vi "Main.vi"(10 "IP":string, 11 "Module Admin":refnum<class "Delacor_lib_QMH_Cloneable Module Admin.lvclass">) -> ()   [LabVIEW 2026, in "My Cloneable Module.lvlib"]
doc: "This template is based off of the Queued Message Handler design pattern and the Queued Message Handler project template that ships with LabVIEW.\n\nThe main difference is that the queue is private to this module and communication between modules is performed via Broadcast and Request events.\n\nRequest events are wrapped in public API methods and are handled in the Event Handling Loop (EHL) of this VI. Any module can register for Broadcast events sent by this module. The EHL generates messages based on user interface actions.\n\nThe Message Handling Loop (MHL) processes messages generated by the EHL, or by other messages. The messages are string values, so new messages can be added easily to the Message Cases case structure in the MHL. Each message cluster can also provide an optional value for Message Data, which is a variant that can be converted to whatever message-specific data is required.\n_____\nBased on DQMH Dev Tools: Project Template 7.1.2.1547."
uses:
  My Cloneable Module.lvlib
  <vilib>/Delacor/Delacor QMH/Libraries/Cloneable Module Admin_class/Delacor_lib_QMH_Cloneable Module Admin.lvclass
  C:/Program Files/National Instruments/LabVIEW 2026/vi.lib/Delacor/Delacor QMH/Libraries/Module Admin_class/Delacor_lib_QMH_Module Admin.lvclass
  Module Data--cluster.ctl
  Do Something Argument--cluster.ctl
  <vilib>/Delacor/Delacor QMH/Libraries/Cloneable Module Admin_class/Delacor_lib_QMH_Cloneable Module Admin.lvclass/Delacor_lib_QMH_Cloneable Module Admin.ctl
  <vilib>/Delacor/Delacor QMH/Libraries/Message Queue_class/Delacor_lib_QMH_Message Queue.lvclass/Delacor_lib_QMH_Message Queue.ctl
  Do Something Else Argument--cluster.ctl
  Do Something Else and Wait for Reply Argument--cluster.ctl
  Do Something Else and Wait (Reply Payload)--cluster.ctl
  Stop Argument--cluster.ctl
  <vilib>/Delacor/Delacor QMH/Libraries/Module Admin_class/Delacor_lib_QMH_Module Admin.lvclass/Delacor_lib_QMH_Module Admin.ctl
  <vilib>/Utility/miscctls.llb/LVPointTypeDef.ctl
  <vilib>/Delacor/Delacor QMH/Libraries/Message Queue_class/Delacor_lib_QMH_Enqueue Message (Single).vi
  <vilib>/Delacor/Delacor QMH/Libraries/Cloneable Module Admin_class/Delacor_lib_QMH_Get Module ID.vi
  <vilib>/Delacor/Delacor QMH/Libraries/Module Admin_class/Delacor_lib_QMH_Get External Launch.vi
  <vilib>/Delacor/Delacor QMH/Libraries/Message Queue_class/Delacor_lib_QMH_Message Queue.lvclass
panel:
  out "error out":errorcluster
  out "X":dbl
  out "Status":string
  in  "Simulate EHL Error":bool
  in  "Simulate MHL Error":bool
  in  "Do Something Else <Replace Me>":bool
  in  "Do Something <Replace Me>":bool
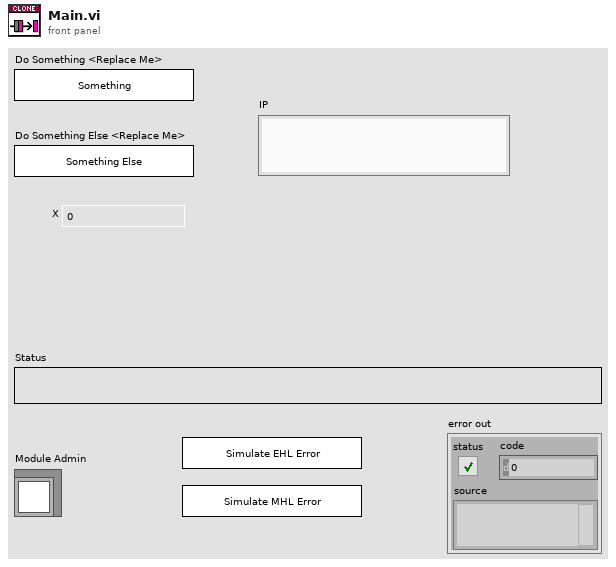
[diagram p1: front panel]
types:
  T1 = typedef "My Cloneable Module.lvlib/Request Events--cluster.ctl" = cluster{"Stop Module":refnum<user-event>, "Do Something":refnum<user-event>, "Do Something Else":refnum<user-event>, "Do Something Else and Wait for Reply":refnum<user-event>, "Show Panel":refnum<user-event>, "Hide Panel":refnum<user-event>, "Show Diagram":refnum<user-event>, "Get Module Execution Status":refnum<user-event>, "Request a HL":refnum<user-event>}
  T2 = typedef "My Cloneable Module.lvlib/Module Data--cluster.ctl" = cluster{"Status":string}
  T3 = typedef "My Cloneable Module.lvlib/Do Something Argument--cluster.ctl" = cluster{"Module ID":i32, "Do Something Msg":string}
  T4 = typedef "My Cloneable Module.lvlib/Do Something Else Argument--cluster.ctl" = cluster{"Module ID":i32, "Do Something Else Msg":string, "X":dbl}
  T5 = typedef "My Cloneable Module.lvlib/Do Something Else and Wait for Reply Argument--cluster.ctl" = cluster{"Module ID":i32, "Do Something Else Msg":string, "X":dbl, "Wait Notifier":refnum<notifier>, "wait for reply":bool}
  T6 = enum32{"invalid lock state", "Not Locked", "Locked (No Password)", "Password-protected"}
  T7 = typedef "My Cloneable Module.lvlib/Stop Argument--cluster.ctl" = cluster{"Module ID":i32, "Origin":string, "Exit via Stop Module Req?":bool, "Wait for Module to stop?":bool}
  T8 = typedef "LVPointTypeDef.ctl" = cluster{"Horizontal":i16, "Vertical":i16}
  T9 = enum32{"Invalid", "Standard", "Closed", "Hidden", "Minimized", "Maximized"}
  T10 = typedef "My Cloneable Module.lvlib/Do Something Else and Wait (Reply Payload)--cluster.ctl" = cluster{"Value":dbl, "error":errorcluster, "Module ID":i32}
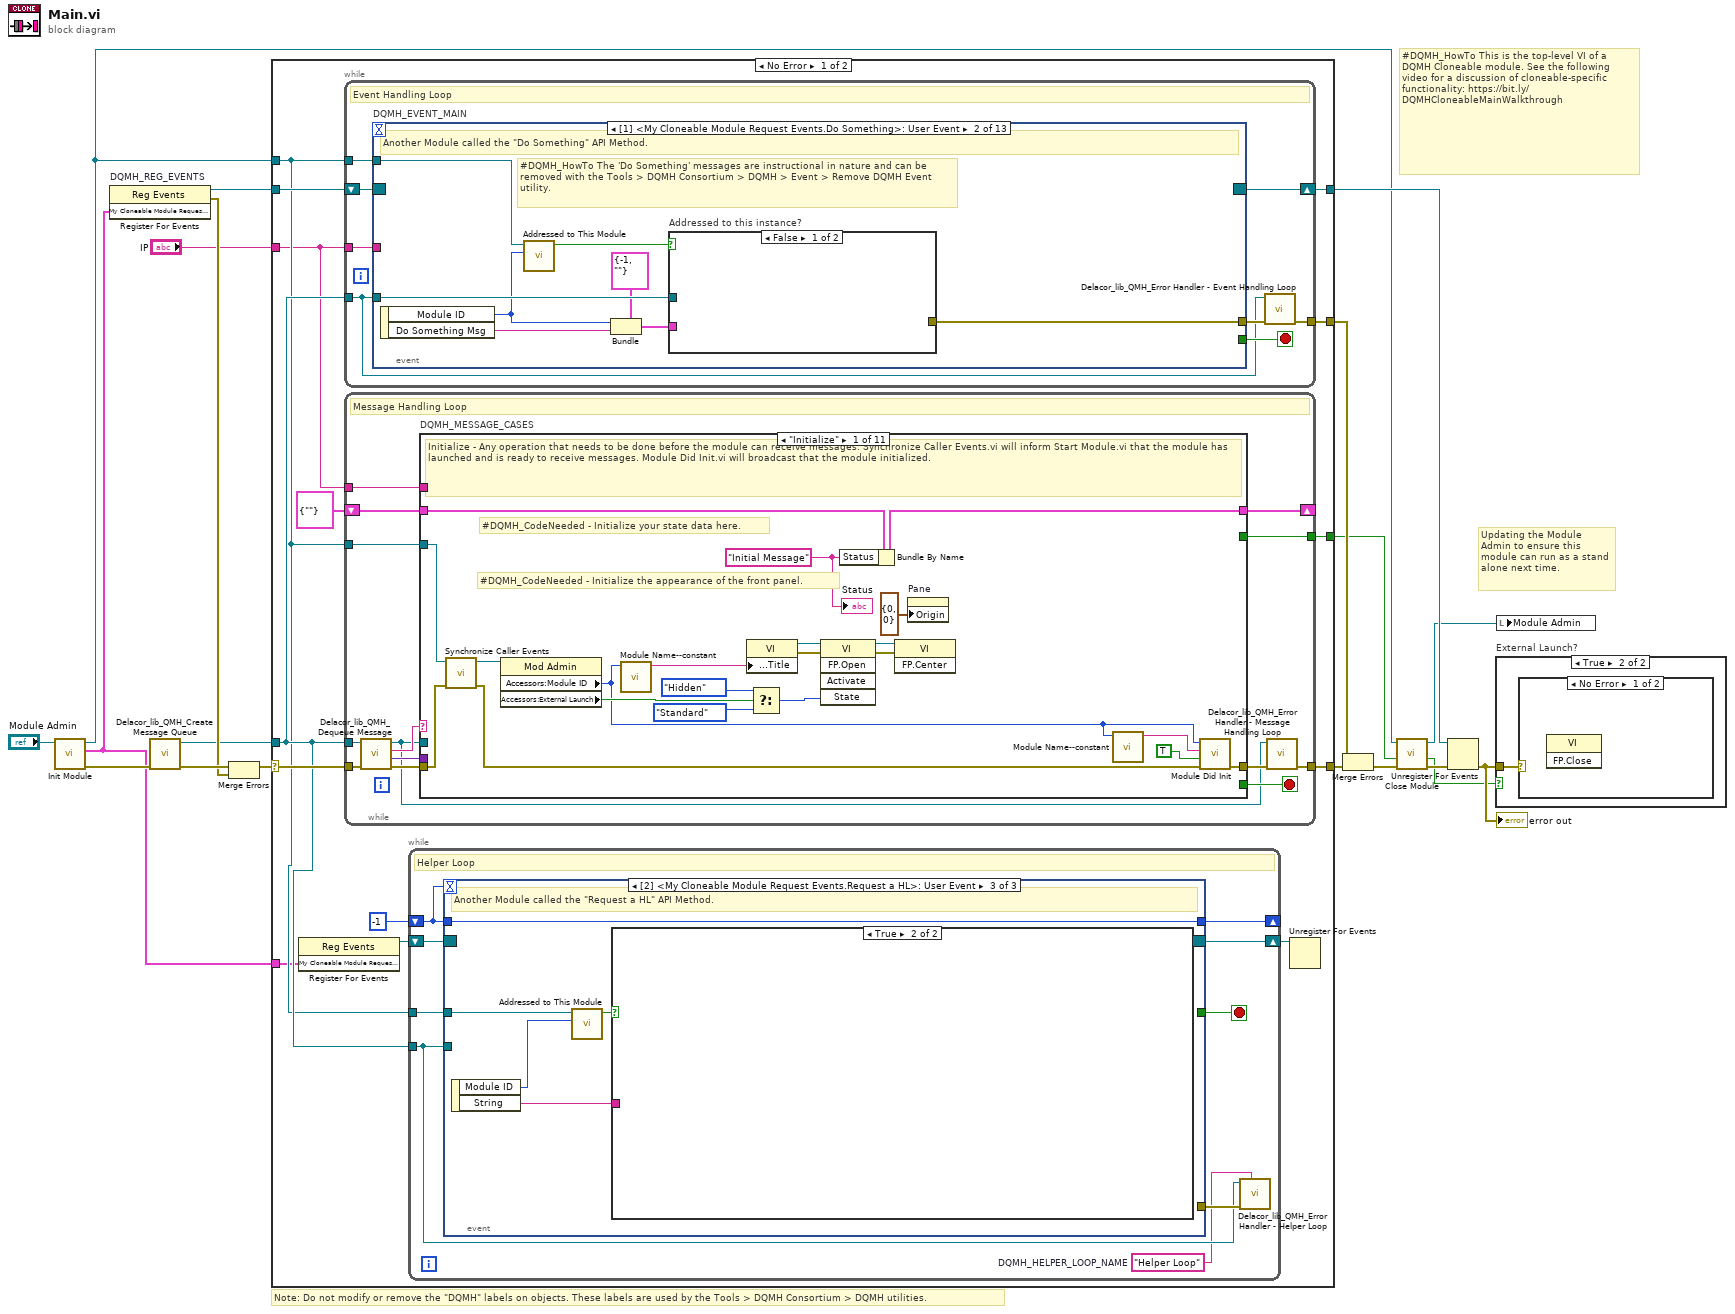
[diagram p0: block diagram]
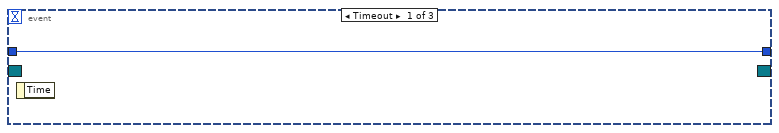
[diagram p2: hidden frame]
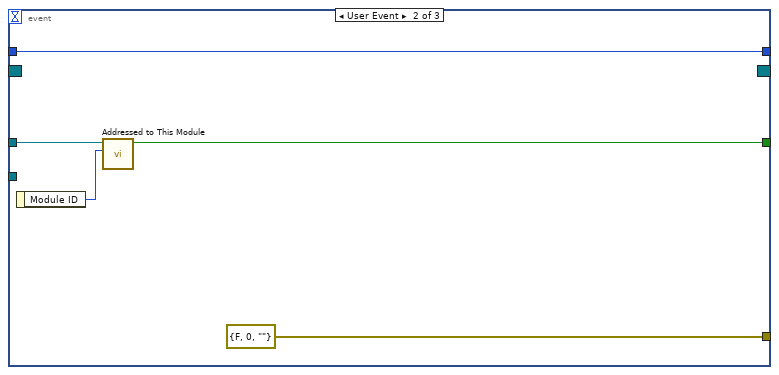
[diagram p3: hidden frame]
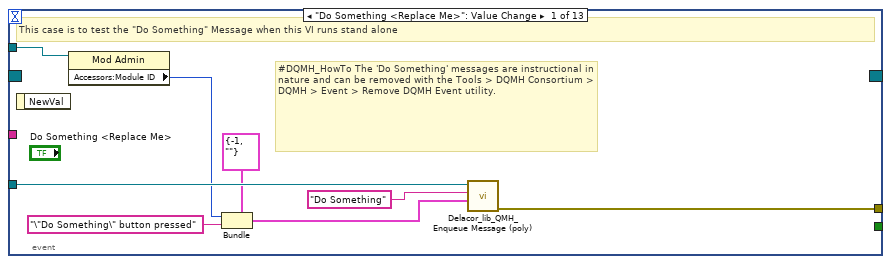
[diagram p5: hidden frame]
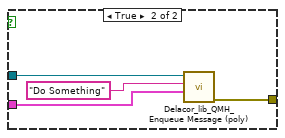
[diagram p6: hidden frame]
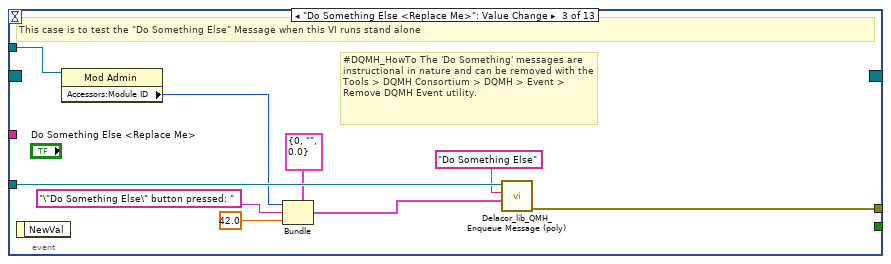
[diagram p7: hidden frame]
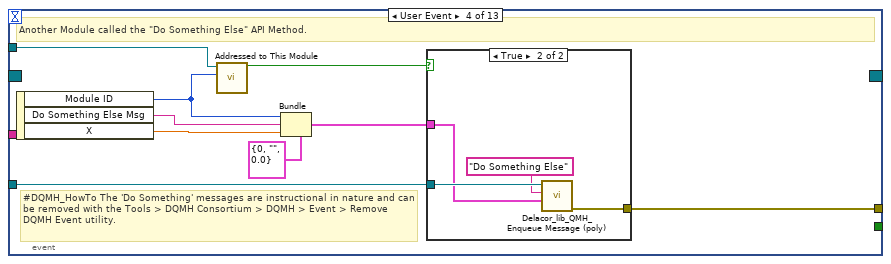
[diagram p8: hidden frame]
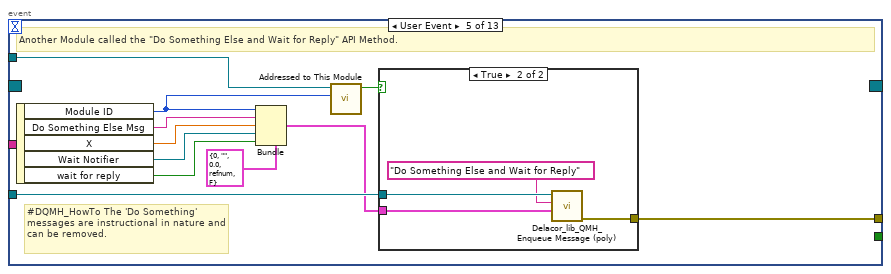
[diagram p10: hidden frame]
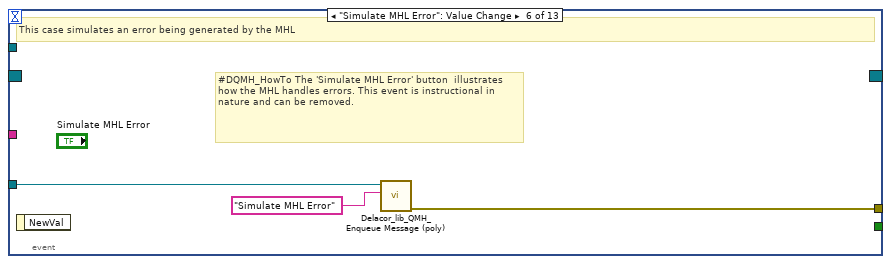
[diagram p12: hidden frame]
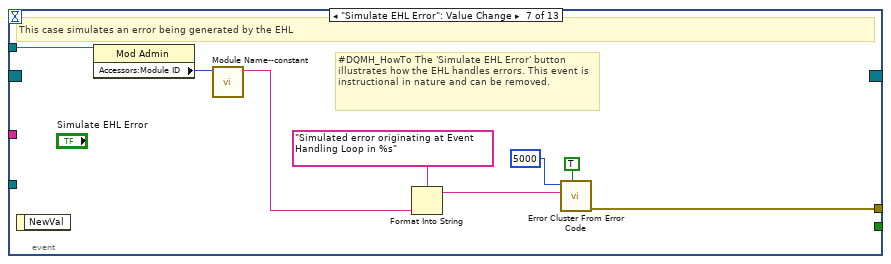
[diagram p13: hidden frame]
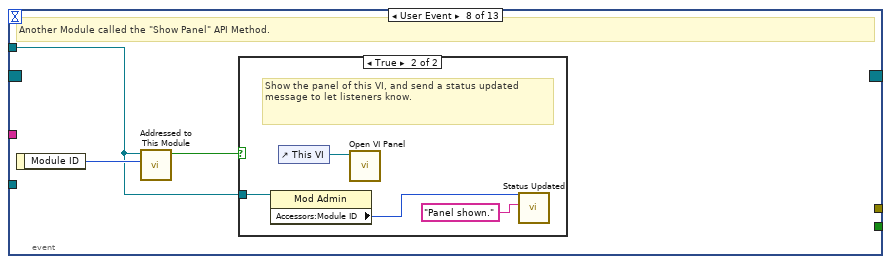
[diagram p14: hidden frame]
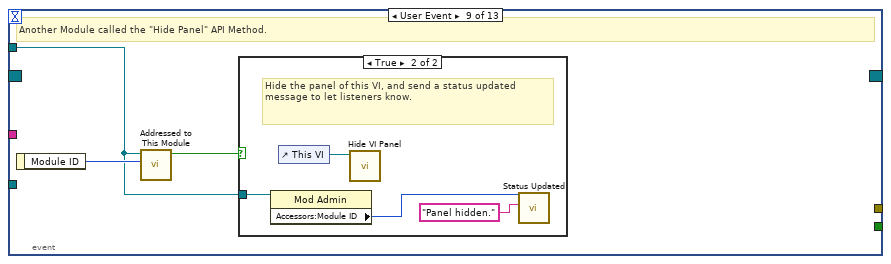
[diagram p16: hidden frame]
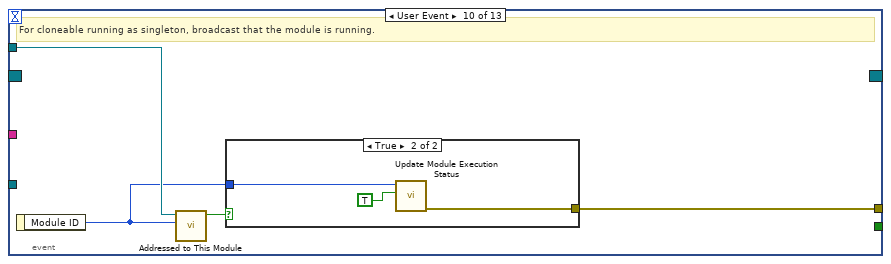
[diagram p18: hidden frame]
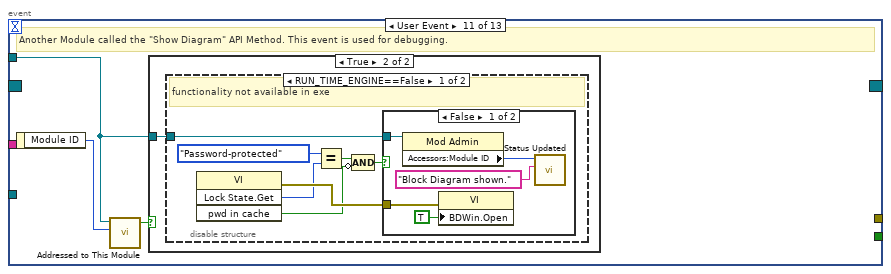
[diagram p20: hidden frame]
diagram:
  # "#DQMH_HowTo This is the top-level VI of a DQMH Cloneable module. See the following video for a discussion of cloneable-specific functionality: https://bit.ly/DQMHCloneableMainWalkthrough"
  # "Note: Do not modify or remove the \"DQMH\" labels on objects. These labels are used by the Tools > DQMH Consortium > DQMH utilities."
  # "Updating the Module Admin to ensure this module can run as a stand alone next time."
  n1 = call "Init Module.vi"("Cloneable Module Admin in"="Module Admin") -> ("error out"=w16:errorcluster, "My Cloneable Module Request Events"=w1:T1, "Cloneable Module Admin out"=w6:refnum<class "Delacor_lib_QMH_Cloneable Module Admin.lvclass">)  [unwired: 8 in]
  n2 = register-events "DQMH_REG_EVENTS"(w1) -> (reference out=w9:refnum<event-registration>, error out=w11:errorcluster)  [unwired: 2 in]
  n3 = call <vilib>:"Delacor_lib_QMH_Create Message Queue.vi"("error in"=w16) -> ("error out"=w13:errorcluster, "Message Queue"=w8:refnum<class "Delacor_lib_QMH_Message Queue.lvclass">)  [unwired: 9 in]
  n4 = Merge Errors(w13, w11) -> (w12:errorcluster)
  n5 = case shown="No Error" w12 {
    selector: w12 -> [w31 w364]
    tunnel: [w33 w363] -> w17
    tunnel: [w30 w362] -> w10
    tunnel: w9 -> [w28 w362]
    tunnel: w8 -> [w27 w355]
    tunnel: [w32 _] -> w18
    tunnel: w6 -> [w26 w358]
    tunnel: [w25 _] -> w4
    tunnel: "IP" -> [w24 _]
    tunnel: w1 -> [w23 _]
    frame No Error {
      n6 = register-events ("DQMH_HELPER_REGFOREVENTS")(w23) -> (reference out=w21:refnum<event-registration>)  [unwired: 2 in, 1 out]
      n7 = while {
        tunnel: w27 -> [w55]
        shift-right: [w58] -> w30
        shift-left: w28 -> [w59]
        tunnel: [w60] -> w32
        tunnel: w26 -> [w56]
        tunnel: w24 -> [w54]
        stop <- w57 stop-if-true
        # "Event Handling Loop"
        n8 = event "DQMH_EVENT_MAIN" shown="[1] <My Cloneable Module Request Events.Do Something>: User Event" {
          selector: w59 -> [_ _ _ _ _ _ _ _ _ _ _ _ _]
          dyn-events: [_ _ _ _ _ _ _ _ _ _ _ _ _] -> w58
          timeout: _ -> [_ _ _ _ _ _ _ _ _ _ _ _ _]
          tunnel: [_ _ _ _ _ _ _ _ _ _ _ w170 _] -> w57
          tunnel: w55 -> [w68 w76 w89 w98 w113 w120 _ _ _ _ _ w173 w190]
          tunnel: [w69 w77 w90 w99 w114 w121 w129 _ _ w147 _ w174 w193] -> w61
          tunnel: w56 -> [w64 w74 w83 w96 w111 _ w128 w130 w137 w145 w151 w172 w191]
          tunnel: w54 -> [_ _ _ _ _ _ _ _ _ _ _ _ _]
          event "Do Something <Replace Me>": Value Change {
            # "#DQMH_HowTo The 'Do Something' messages are instructional in nature and can be removed with the Tools > DQMH Consortium > DQMH > Event > Remove DQMH Event utility."
            # "This case is to test the \"Do Something\" Message when this VI runs stand alone"
            n9 = event-data() -> ()  [unwired: 1 in, 1 out]
            n10 = property on="Property Node" class="Mod Admin"(reference=w64) -> ("Accessors:Module ID"=w63:i32)  [unwired: 1 in, 2 out]
            n11 = Bundle(cluster=T3 {"Module ID"=-1, "Do Something Msg"=""} ("Do Something Argument"), "Module ID"=w63, "Do Something Msg"="\"Do Something\" button pressed" ("\"Do Something\" button pressed")) -> (w66:T3)
            n12 = call-poly <vilib>:"Delacor_lib_QMH_Enqueue Message (poly).vi"("Message Data"=w66, "Message"="Do Something", "Message Queue in"=w68) -> ("error out"=w69:errorcluster)  [unwired: 7 in, 1 out]
          }
          event User Event {
            # "#DQMH_HowTo The 'Do Something' messages are instructional in nature and can be removed with the Tools > DQMH Consortium > DQMH > Event > Remove DQMH Event utility."
            # "Another Module called the \"Do Something\" API Method."
            n13 = event-data() -> ("Module ID"=w71:i32, "Do Something Msg"=w70:string)  [unwired: 1 in]
            n14 = call "Addressed to This Module.vi"("Module ID from Argument"=w71, "Module Admin"=w74) -> ("Addressed to this instance?"=w75:bool)  [unwired: 8 in, 1 out]
            n15 = Bundle(cluster=T3 {"Module ID"=-1, "Do Something Msg"=""} ("Do Something Argument"), "Module ID"=w71, "Do Something Msg"=w70) -> (w73:T3)
            n16 = case "Addressed to this instance?" shown="False" w75 {
              tunnel: w76 -> [_ w80]
              tunnel: [_ w81] -> w77
              tunnel: w73 -> [_ w78]
              frame False {
                # "Do nothing"
              }
              frame True {
                n17 = call-poly <vilib>:"Delacor_lib_QMH_Enqueue Message (poly).vi"("Message Data"=w78, "Message"="Do Something", "Message Queue in"=w80) -> ("error out"=w81:errorcluster)  [unwired: 7 in, 1 out]
              }
            }
          }
          event "Do Something Else <Replace Me>": Value Change {
            # "#DQMH_HowTo The 'Do Something' messages are instructional in nature and can be removed with the Tools > DQMH Consortium > DQMH > Event > Remove DQMH Event utility."
            # "This case is to test the \"Do Something Else\" Message when this VI runs stand alone"
            n18 = event-data() -> ()  [unwired: 1 in, 1 out]
            n19 = property on="Property Node" class="Mod Admin"(reference=w83) -> ("Accessors:Module ID"=w82:i32)  [unwired: 1 in, 2 out]
            n20 = Bundle(cluster=T4 {"Module ID"=0, "Do Something Else Msg"="", "X"=0.0} ("Do Something Else Argument"), "Module ID"=w82, "Do Something Else Msg"="\"Do Something Else\" button pressed: " ("\"Do Something Else\" button pressed"), "X"=42.0) -> (w86:T4)
            n21 = call-poly <vilib>:"Delacor_lib_QMH_Enqueue Message (poly).vi"("Message Data"=w86, "Message"="Do Something Else", "Message Queue in"=w89) -> ("error out"=w90:errorcluster)  [unwired: 7 in, 1 out]
          }
          event User Event {
            # "#DQMH_HowTo The 'Do Something' messages are instructional in nature and can be removed with the Tools > DQMH Consortium > DQMH > Event > Remove DQMH Event utility."
            # "Another Module called the \"Do Something Else\" API Method."
            n22 = event-data() -> ("Module ID"=w91:i32, "Do Something Else Msg"=w92:string, "X"=w94:dbl)  [unwired: 1 in]
            n23 = call "Addressed to This Module.vi"("Module ID from Argument"=w91, "Module Admin"=w96) -> ("Addressed to this instance?"=w97:bool)  [unwired: 8 in, 1 out]
            n24 = Bundle(cluster=T4 {"Module ID"=0, "Do Something Else Msg"="", "X"=0.0} ("Do Something Else Argument"), "Module ID"=w91, "Do Something Else Msg"=w92, "X"=w94) -> (w93:T4)
            n25 = case shown="True" w97 {
              tunnel: w98 -> [_ w102]
              tunnel: [_ w103] -> w99
              tunnel: w93 -> [_ w100]
              frame False {
              }
              frame True {
                n26 = call-poly <vilib>:"Delacor_lib_QMH_Enqueue Message (poly).vi"("Message Data"=w100, "Message"="Do Something Else", "Message Queue in"=w102) -> ("error out"=w103:errorcluster)  [unwired: 7 in, 1 out]
              }
            }
          }
          event User Event {
            # "#DQMH_HowTo The 'Do Something' messages are instructional in nature and can be removed."
            # "Another Module called the \"Do Something Else and Wait for Reply\" API Method."
            n27 = event-data() -> ("Module ID"=w109:i32, "Do Something Else Msg"=w107:string, "X"=w106:dbl, "Wait Notifier"=w105:refnum<notifier>, "wait for reply"=w104:bool)  [unwired: 1 in]
            n28 = Bundle(cluster=T5 {"Module ID"=0, "Do Something Else Msg"="", "X"=0.0, "Wait Notifier"=refnum, "wait for reply"=FALSE} ("Do Something Else and Wait for Reply Argument"), "Module ID"=w109, "Do Something Else Msg"=w107, "X"=w106, "Wait Notifier"=w105, "wait for reply"=w104) -> (w108:T5)
            n29 = call "Addressed to This Module.vi"("Module ID from Argument"=w109, "Module Admin"=w111) -> ("Addressed to this instance?"=w112:bool)  [unwired: 8 in, 1 out]
            n30 = case shown="True" w112 {
              tunnel: [_ w118] -> w114
              tunnel: w113 -> [_ w117]
              tunnel: w108 -> [_ w115]
              frame False {
              }
              frame True {
                n31 = call-poly <vilib>:"Delacor_lib_QMH_Enqueue Message (poly).vi"("Message Data"=w115, "Message"="Do Something Else and Wait for Reply", "Message Queue in"=w117) -> ("error out"=w118:errorcluster)  [unwired: 7 in, 1 out]
              }
            }
          }
          event "Simulate MHL Error": Value Change {
            # "#DQMH_HowTo The 'Simulate MHL Error' button  illustrates how the MHL handles errors. This event is instructional in nature and can be removed."
            # "This case simulates an error being generated by the MHL"
            n32 = event-data() -> ()  [unwired: 1 in, 1 out]
            n33 = call-poly <vilib>:"Delacor_lib_QMH_Enqueue Message (poly).vi"("Message"="Simulate MHL Error", "Message Queue in"=w120) -> ("error out"=w121:errorcluster)  [unwired: 8 in, 1 out]
          }
          event "Simulate EHL Error": Value Change {
            # "#DQMH_HowTo The 'Simulate EHL Error' button  illustrates how the EHL handles errors. This event is instructional in nature and can be removed."
            # "This case simulates an error being generated by the EHL"
            n34 = event-data() -> ()  [unwired: 1 in, 1 out]
            n35 = property on="Property Node" class="Mod Admin"(reference=w128) -> ("Accessors:Module ID"=w127:i32)  [unwired: 1 in, 2 out]
            n36 = call "Module Name--constant.vi"("Module ID"=w127) -> ("Module Name"=w122:string)  [unwired: 10 in]
            n37 = Format Into String(format string="Simulated error originating at Event Handling Loop in %s", w122) -> (resulting string=w125:string)  [unwired: 2 in, 1 out]
            n38 = call <vilib>:"Error Cluster From Error Code.vi"("show call chain? (False)"=TRUE, "error message (\"\")"=w125, "error code (0)"=5000) -> ("error out"=w129:errorcluster)  [unwired: 6 in]
          }
          event User Event {
            # "Another Module called the \"Show Panel\" API Method."
            n39 = event-data() -> ("Module ID"=w131:i32)  [unwired: 1 in]
            n40 = call "Addressed to This Module.vi"("Module ID from Argument"=w131, "Module Admin"=w130) -> ("Addressed to this instance?"=w132:bool)  [unwired: 8 in, 1 out]
            n41 = case shown="True" w132 {
              tunnel: w130 -> [_ w134]
              frame False {
              }
              frame True {
                # "Show the panel of this VI, and send a status updated message to let listeners know."
                n42 = property on="Property Node" class="Mod Admin"(reference=w134) -> ("Accessors:Module ID"=w133:i32)  [unwired: 1 in, 2 out]
                n43 = control-ref of="This VI"() -> (w136:refnum<vi>)
                n44 = call "Open VI Panel.vi"("VI"=w136) -> ()  [unwired: 10 in, 1 out]
                n45 = call "Status Updated.vi"("Status"="Panel shown." ("format string"), "Module ID"=w133) -> ()  [unwired: 9 in, 1 out]
              }
            }
          }
          event User Event {
            # "Another Module called the \"Hide Panel\" API Method."
            n46 = event-data() -> ("Module ID"=w138:i32)  [unwired: 1 in]
            n47 = call "Addressed to This Module.vi"("Module ID from Argument"=w138, "Module Admin"=w137) -> ("Addressed to this instance?"=w139:bool)  [unwired: 8 in, 1 out]
            n48 = case shown="True" w139 {
              tunnel: w137 -> [_ w141]
              frame False {
              }
              frame True {
                # "Hide the panel of this VI, and send a status updated message to let listeners know."
                n49 = property on="Property Node" class="Mod Admin"(reference=w141) -> ("Accessors:Module ID"=w140:i32)  [unwired: 1 in, 2 out]
                n50 = control-ref of="This VI"() -> (w143:refnum<vi>)
                n51 = call "Hide VI Panel.vi"("VI"=w143) -> ()  [unwired: 10 in, 1 out]
                n52 = call "Status Updated.vi"("Status"="Panel hidden." ("format string"), "Module ID"=w140) -> ()  [unwired: 9 in, 1 out]
              }
            }
          }
          event User Event {
            # "For cloneable running as singleton, broadcast that the module is running."
            n53 = event-data() -> ("Module ID"=w144:i32)  [unwired: 1 in]
            n54 = call "Addressed to This Module.vi"("Module ID from Argument"=w144, "Module Admin"=w145) -> ("Addressed to this instance?"=w146:bool)  [unwired: 8 in, 1 out]
            n55 = case shown="True" w146 {
              tunnel: [_ w150] -> w147
              tunnel: w144 -> [_ w149]
              frame False {
              }
              frame True {
                n56 = call "Update Module Execution Status.vi"("Running?"=TRUE, "Module ID"=w149) -> ("error out"=w150:errorcluster)  [unwired: 9 in]
              }
            }
          }
          event User Event {
            # "Another Module called the \"Show Diagram\" API Method. This event is used for debugging."
            n57 = event-data() -> ("Module ID"=w152:i32)  [unwired: 1 in]
            n58 = call "Addressed to This Module.vi"("Module ID from Argument"=w152, "Module Admin"=w151) -> ("Addressed to this instance?"=w153:bool)  [unwired: 8 in, 1 out]
            n59 = case shown="True" w153 {
              tunnel: w151 -> [_ w154]
              frame False {
              }
              frame True {
                n60 = disable-structure shown="RUN_TIME_ENGINE==False" {
                  disable-tunnel: w154 -> [w155 _]
                  frame condition #0 (active) {
                    # "functionality not available in exe"
                    n61 = invoke on="Invoke Node" class="VI" method="Lock State.Get"() -> (error out=w161:errorcluster, "Get Lock State"=w160:T6, "pwd in cache"=w157:bool)  [unwired: 4 in, 1 out]
                    n62 = Equal?(x=T6."Password-protected", y=w160) -> (x = y?=w158:bool)
                    n63 = Compound Arithmetic op=AND(w158, invert w157) -> (w156:bool)
                    n64 = case shown="False" w156 {
                      tunnel: w161 -> [w166 _]
                      tunnel: w155 -> [w163 _]
                      frame False {
                        n65 = property on="Property Node" class="Mod Admin"(reference=w163) -> ("Accessors:Module ID"=w162:i32)  [unwired: 1 in, 2 out]
                        n66 = property on="Property Node" class="VI"(error in=w166, "BDWin.Open"=TRUE ("Block Diagram Window:Open")) -> ()  [unwired: 1 in, 2 out]
                        n67 = call "Status Updated.vi"("Status"="Block Diagram shown." ("format string"), "Module ID"=w162) -> ()  [unwired: 9 in, 1 out]
                      }
                      frame True {
                        # "Password-protected VI, and the password is not in the cache. Do not show the diagram."
                      }
                    }
                  }
                  frame condition #1 {
                  }
                }
              }
            }
          }
          event User Event {
            # "Another Module called the \"Stop Module\" API Method  or the Message Handling Loop below."
            n68 = event-data() -> ("Module ID"=w168:i32, "Wait for Module to stop?"=w169:bool, "Origin"=w167:string)  [unwired: 1 in]
            n69 = call "Addressed to This Module.vi"("Module ID from Argument"=w168, "Module Admin"=w172) -> ("Addressed to this instance?"=w171:bool)  [unwired: 8 in, 1 out]
            n70 = case shown="True" w171 {
              tunnel: [_ w186] -> w174
              tunnel: w173 -> [_ w182]
              tunnel: [_ TRUE] -> w170
              tunnel: w169 -> [_ w177]
              tunnel: w168 -> [_ w179]
              tunnel: w167 -> [_ w175]
              frame False {
              }
              frame True {
                # "The event can get fired from the Exit message. The queue gets destroyed there. In this case, the Enqueue VI will return error 1. It is safe to ignore, because the module is already exiting."
                n71 = local write "Status"(w175) -> ()
                n72 = Bundle By Name(cluster=T7 {"Module ID"=-1, "Origin"="", "Exit via Stop Module Req?"=FALSE, "Wait for Module to stop?"=FALSE} ("Stop Argument"), "Module ID"=w179, "Exit via Stop Module Req?"=TRUE, "Wait for Module to stop?"=w177) -> (w176:T7)
                n73 = call-poly <vilib>:"Delacor_lib_QMH_Enqueue Message (poly).vi"("Priority Message? (F)"=TRUE, "Message Data"=w176, "Message"="Exit", "Message Queue in"=w182) -> ("error out"=w187:errorcluster)  [unwired: 6 in, 1 out]
                n74 = call <vilib>:"Clear Errors.vi"("error in (no error)"=w187, "specific error code to clear (0: all)"=1) -> ("error out"=w186:errorcluster)  [unwired: 4 in, 1 out]
              }
            }
          }
          event Panel Close? {
            w192 = TRUE  # Discard the event, the MHL is responsible for closing and stopping this VI.
            # "Hide the panel or send the 'Exit' message if the user clicks the 'X' on the module main VI panel."
            n75 = event-data() -> ()  [unwired: 1 in, 1 out]
            n76 = property on="Property Node" class="Mod Admin"(reference=w191) -> (reference out=w188:refnum<class "Delacor_lib_QMH_Cloneable Module Admin.lvclass">, "Accessors:External Launch"=w189:bool)  [unwired: 1 in, 1 out]
            n77 = case shown="True" w189 {
              tunnel: w190 -> [_ w201]
              tunnel: [_ w202] -> w193
              tunnel: w188 -> [w196 _]
              frame True {
                # "If externally launched, clicking the 'X' hides the panel, but doesn't close it."
                n78 = property on="Property Node" class="Mod Admin"(reference=w196) -> ("Accessors:Module ID"=w195:i32)  [unwired: 1 in, 2 out]
                n79 = call "Status Updated.vi"("Status"="Panel hidden." ("format string"), "Module ID"=w195) -> ("error out"=w194:errorcluster)  [unwired: 9 in]
                n80 = control-ref of="This VI"() -> (w198:refnum<vi>)
                n81 = call "Hide VI Panel.vi"("error in"=w194, "VI"=w198) -> ()  [unwired: 9 in, 1 out]
              }
              frame False {
                # "If run as a stand-alone VI, clicking the panel 'X' stops the VI."
                n82 = call-poly <vilib>:"Delacor_lib_QMH_Enqueue Message (poly).vi"("Priority Message? (F)"=TRUE, "Message"="Exit", "Message Queue in"=w201) -> ("error out"=w202:errorcluster)  [unwired: 7 in, 1 out]
              }
            }
            n83 = event-data ("Event Filter Node")("Discard?"=w192) -> ()  [unwired: 1 in, 1 out]
          }
        }
        n84 = call-dynamic "Delacor_lib_QMH_Error Handler - Event Handling Loop.vi"("error in"=w61, "Message Queue in"=w55) -> ("dup error in"=w60:errorcluster)  [unwired: 8 in, 1 out]
      }
      n85 = while {
        tunnel: w27 -> [w204]
        shift-right: [w211] -> _
        shift-left: T2 {"Status"=""} ("Data Cluster") -> [w212]
        tunnel: w31 -> [w215]
        tunnel: [w213] -> w33
        tunnel: w26 -> [w206]
        tunnel: [w205] -> w25
        tunnel: w24 -> [w203]
        stop <- w210 stop-if-true
        # "Message Handling Loop"
        n86 = call-dynamic "Delacor_lib_QMH_Dequeue Message.vi"("error in"=w215, "Message Queue in"=w204) -> ("error out"=w214:errorcluster, "Message Data"=w208:variant, "Message"=w209:string, "Message Queue out"=w207:refnum<class "Delacor_lib_QMH_Message Queue.lvclass">)  [unwired: 6 in]
        n87 = case "DQMH_MESSAGE_CASES" shown="\"Initialize\"" w209 {
          selector: w209 -> [_ _ _ _ _ _ _ _ _ _ w344]
          tunnel: w207 -> [_ _ _ _ _ _ _ w299 _ w336 _]
          tunnel: w214 -> [w235 w239 w249 w260 w281 w294 w296 w308 w325 w342 w353]
          tunnel: [w233 w239 w247 w259 w280 w293 w296 w304 w324 w337 w354] -> w216
          tunnel: w212 -> [w226 w238 w246 w258 w261 w292 w295 w303 w322 w335 w351]
          tunnel: [w225 w238 w246 w258 w261 w292 w295 w303 w322 w335 w351] -> w211
          tunnel: [_ _ _ _ _ _ _ _ _ w334 _] -> w210
          tunnel: w208 -> [_ _ w245 w255 w275 _ _ w302 _ w332 _]
          tunnel: w206 -> [w221 _ w241 w251 w266 _ _ w301 w320 w327 w350]
          tunnel: [_ _ _ _ _ _ _ _ _ w330 _] -> w205
          tunnel: w203 -> [_ _ _ _ _ _ _ _ _ _ _]
          frame "Initialize" {
            w218 = "Initial Message" ("Initial Message")
            # "#DQMH_CodeNeeded - Initialize the appearance of the front panel."
            # "#DQMH_CodeNeeded - Initialize your state data here."
            # "Initialize - Any operation that needs to be done before the module can receive messages. Synchronize Caller Events.vi will inform Start Module.vi that the module has launched and is ready to receive messages. Module Did Init.vi will broadcast that the module initialized."
            n88 = call "Synchronize Caller Events.vi"("error in"=w235, "Module Admin"=w221) -> ("error out"=w234:errorcluster, "Module Admin out"=w220:refnum<class "Delacor_lib_QMH_Cloneable Module Admin.lvclass">)  [unwired: 8 in]
            n89 = property on="Property Node" class="Mod Admin"(reference=w220) -> ("Accessors:Module ID"=w217:i32, "Accessors:External Launch"=w222:bool)  [unwired: 1 in, 2 out]
            n90 = call "Module Name--constant.vi"("Module ID"=w217) -> ("Module Name"=w230:string)  [unwired: 10 in]
            n91 = property on="Property Node" class="VI"("Front Panel.Title"=w230) -> (reference out=w232:refnum<vi>, error out=w237:errorcluster)  [unwired: 2 in]
            n92 = Select(t=T9."Hidden" ("State"), s=w222, f=T9."Standard" ("State")) -> (s? t:f=w227:T9)
            n93 = invoke on="Invoke Node" class="VI" method="FP.Open"(reference=w232, error in=w237, "State"=w227) -> (reference out=w231:refnum<vi>, error out=w236:errorcluster)  [unwired: 2 in, 3 out]
            n94 = Bundle By Name(cluster=w226, "Status"=w218) -> (w225:T2)
            n95 = invoke on="Invoke Node" class="VI" method="FP.Center"(reference=w231, error in=w236) -> ()  [unwired: 1 in, 3 out]
            n96 = property on="Pane" class="Pane"("Origin"=T8 {"Horizontal"=0, "Vertical"=0}) -> ()  [unwired: 2 in, 2 out]
            n97 = call "Module Name--constant.vi"("Module ID"=w217) -> ("Module Name"=w223:string)  [unwired: 10 in]
            n98 = call "Module Did Init.vi"("error in"=w234, "Initialized?"=TRUE, "Origin"=w223, "Module ID"=w217) -> ("error out"=w233:errorcluster)  [unwired: 7 in]
            "Status" <- w218
          }
          frame "---Module Specific---" {
            # "Separator -- The following cases handle messages specific to this Module."
          }
          frame "Do Something" {
            # "#DQMH_HowTo The 'Do Something' messages are instructional in nature and can be removed with the Tools > DQMH Consortium > DQMH > Event > Remove DQMH Event utility."
            # "Do Something - Replace this message with functionality for your own application. Note that this message also fires the \"Did Something\" broadcast event."
            n99 = Variant To Data(error in=w249, type=T3 {"Module ID"=-1, "Do Something Msg"=""} ("Do Something Argument"), Variant=w245) -> (data=w244:T3, error out=w248:errorcluster)
            n100 = property on="Property Node" class="Mod Admin"(reference=w241) -> ("Accessors:Module ID"=w240:i32)  [unwired: 1 in, 2 out]
            n101 = Unbundle By Name(w244) -> ("Do Something Msg"=w242:string)
            n102 = call "Status Updated.vi"("Status"=w242, "Module ID"=w240) -> ()  [unwired: 9 in, 1 out]
            n103 = local write "Status"(w242) -> ()
            n104 = call "Did Something.vi"("error in"=w248, "Did Something Msg"=w242, "Module ID"=w240) -> ("error out"=w247:errorcluster)  [unwired: 8 in]
          }
          frame "Do Something Else" {
            # "#DQMH_HowTo The 'Do Something' messages are instructional in nature and can be removed with the Tools > DQMH Consortium > DQMH > Event > Remove DQMH Event utility."
            # "Do Something Else - Replace this message with functionality for your own application."
            n105 = Variant To Data(error in=w260, type=T4 {"Module ID"=0, "Do Something Else Msg"="", "X"=0.0} ("Do Something Else Argument"), Variant=w255) -> (data=w256:T4, error out=w259:errorcluster)
            n106 = Unbundle By Name(w256) -> ("Do Something Else Msg"=w254:string, "X"=w253:dbl)
            "X" <- w253
            n107 = property on="Property Node" class="Mod Admin"(reference=w251) -> ("Accessors:Module ID"=w250:i32)  [unwired: 1 in, 2 out]
            n108 = Format Into String(initial string=w254, w253) -> (resulting string=w252:string)  [unwired: 2 in, 1 out]
            n109 = call "Status Updated.vi"("Status"=w252, "Module ID"=w250) -> ()  [unwired: 9 in, 1 out]
            n110 = local write "Status"(w252) -> ()
          }
          frame "Do Something Else and Wait for Reply" {
            w268 = "X(%.2f)+Offset(%.2f)=%.2f"  # status message format string
            # "#DQMH_HowTo The 'Do Something' messages are instructional in nature and can be removed."
            # "Send back X with a random offset"
            # "Do Something Else and Wait for Reply - Replace this message with functionality for your own application. Note that this message must fire a notifier to let callers know it has finished execution, and it returns an error if the 'Value' is negative."
            n111 = property on="Property Node" class="Mod Admin"(reference=w266) -> ("Accessors:Module ID"=w263:i32)  [unwired: 1 in, 2 out]
            n112 = Variant To Data(error in=w281, type=T5 {"Module ID"=0, "Do Something Else Msg"="", "X"=0.0, "Wait Notifier"=refnum, "wait for reply"=FALSE} ("Do Something Else and Wait for Reply Argument"), Variant=w275) -> (data=w276:T5, error out=w279:errorcluster)
            n113 = Unbundle By Name(w276) -> ("Wait Notifier"=w273:refnum<notifier>, "Do Something Else Msg"=w274:string, "X"=w270:dbl, "wait for reply"=w264:bool)
            n114 = Random Number (0-1)() -> (number: 0 to 1=w269:dbl)
            n115 = Add(x=w269, y=w270) -> (x+y=w265:dbl)
            n116 = Less Than 0?(x=w265) -> (x < 0?=w262:bool)
            n117 = local write "X"(w270) -> ()
            n118 = case shown="True" w262 {
              tunnel: [_ w285] -> w278
              frame False {
              }
              frame True {
                n119 = call <vilib>:"Error Cluster From Error Code.vi"("show call chain? (False)"=TRUE, "error message (\"\")"="The 'Something Else and Wait for Reply' message generated a negative number, which is considered an error condition.", "error code (0)"=5000) -> ("error out"=w285:errorcluster)  [unwired: 6 in]
              }
            }
            n120 = Format Into String(format string=w268, initial string=w274, w270, w269, w265) -> (resulting string=w267:string)  [unwired: 1 in, 1 out]
            n121 = Bundle By Name(cluster=T10 {"Value"=0.0, "error"={"status"=FALSE, "code"=0, "source"=""}, "Module ID"=0} ("notification"), "error"=w278, "Value"=w265, "Module ID"=w263) -> (w271:T10)
            n122 = call "Status Updated.vi"("Status"=w267, "Module ID"=w263) -> ()  [unwired: 9 in, 1 out]
            n123 = local write "Status"(w267) -> ()
            n124 = case shown="True" w264 {
              tunnel: w273 -> [_ w289]
              tunnel: w271 -> [_ w288]
              frame False {
              }
              frame True {
                # "Simulate an operation that requires a wait."
                n125 = flat-sequence {
                  tunnel: w289 -> [w291]
                  tunnel: w288 -> [w290]
                  tunnel: w286 -> [_]
                  frame #0 {
                    n126 = Send Notification(notification=w290, notifier=w291) -> ()  [unwired: 1 in, 2 out]
                  }
                }
                n127 = Wait (ms)(milliseconds to wait=u32 1000) -> (millisecond timer value=w286:u32)
              }
            }
            n128 = Merge Errors(w279, w278) -> (w280:errorcluster)
          }
          frame "---Copy This Frame---" {
            # "Duplicate this frame when creating new messages.  Change this comment in the duplicated frame to describe this message."
            n129 = Merge Errors(w294) -> (w293:errorcluster)
          }
          frame "---Exit and Error Handling---" {
            # "Separator - the following cases handle errors and exit messages."
          }
          frame "Error" {
            # "#DQMH_CodeRecommended - If the module is running in standalone mode (External Launch = FALSE), this code will pop up an error dialog and call the 'Exit' message if an error occurs. Add more fine-grained error management here."
            # "Error - Check the error message data and respond accordingly. This message is sent by the \"Error Handler\" VIs at the end of each loop in this application."
            n130 = property on="Property Node" class="Mod Admin"(reference=w301) -> ("Accessors:External Launch"=w300:bool, "Accessors:Module ID"=w298:i32)  [unwired: 1 in, 2 out]
            n131 = Variant To Data(error in=w308, type=errorcluster {"status"=FALSE, "code"=0, "source"=""} ("error constant"), Variant=w302) -> (data=w297:errorcluster, error out=w306:errorcluster)
            n132 = local write "error out"(w297) -> ()
            n133 = call "Error Reported.vi"("Error"=w297, "Module ID"=w298) -> ()  [unwired: 9 in, 1 out]
            n134 = case shown="False" w300 {
              tunnel: [w313 _] -> w305
              tunnel: w299 -> [w311 _]
              tunnel: w297 -> [w312 _]
              frame False {
                n135 = disable-structure shown="Default" {
                  disable-tunnel: w312 -> [w314 _]
                  frame condition #0 (active) {
                    # "If the module is running standalone, then pop up an error dialog and call the \"Exit\" message."
                    n136 = call <vilib>:"Simple Error Handler.vi"("error in (no error)"=w314) -> ()  [unwired: 4 in, 5 out]
                  }
                  frame condition #1 {
                    # "To prevent the Simple Error Handler VI from being loaded (e.g. when deploying to a Real-Time target), add the Conditional Disable Symbol \"DQMH_Disable_SEH\" to your project and set it to TRUE."
                  }
                }
                n137 = call-poly <vilib>:"Delacor_lib_QMH_Enqueue Message (poly).vi"("Priority Message? (F)"=TRUE, "Message"="Exit", "Message Queue in"=w311) -> ("error out"=w313:errorcluster)  [unwired: 7 in, 1 out]
              }
              frame True {
                # "If the module was launched externally, calling the Error Reported broadcast VI is the only action performed by the \"Error\" message. The module's caller can then process the error appropriately."
              }
            }
            n138 = Merge Errors(w306, w305) -> (w304:errorcluster)
          }
          frame "Simulate MHL Error" {
            # "#DQMH_HowTo The 'Simulate MHL Error' button  illustrates how the MHL handles errors. This event is instructional in nature and can be removed."
            # "Simulate an error occurring at the MHL"
            n139 = property on="Property Node" class="Mod Admin"(reference=w320) -> ("Accessors:Module ID"=w321:i32)  [unwired: 1 in, 2 out]
            n140 = call "Module Name--constant.vi"("Module ID"=w321) -> ("Module Name"=w316:string)  [unwired: 10 in]
            n141 = Format Into String(format string="Simulated error originating at Message Handling Loop in %s", w316) -> (resulting string=w317:string)  [unwired: 2 in, 1 out]
            n142 = call <vilib>:"Error Cluster From Error Code.vi"("show call chain? (False)"=TRUE, "error message (\"\")"=w317, "error code (0)"=5001) -> ("error out"=w323:errorcluster)  [unwired: 6 in]
            n143 = Merge Errors(w325, w323) -> (w324:errorcluster)
          }
          frame "Exit" {
            w333 = 91  # 91: not all Exit messages will have an argument
            w334 = TRUE  # Stop the VI
            # "Release the message queue reference"
            # "#DQMH_CodeNeeded - Add any required cleanup code here."
            # "Exit - Exit the application."
            n144 = Variant To Data(error in=w342, type=T7 {"Module ID"=-1, "Origin"="", "Exit via Stop Module Req?"=FALSE, "Wait for Module to stop?"=FALSE} ("Stop Argument"), Variant=w332) -> (data=w329:T7, error out=w338:errorcluster)
            n145 = call <vilib>:"Clear Errors.vi"("error in (no error)"=w338, "specific error code to clear (0: all)"=w333) -> ("error out"=w341:errorcluster)  [unwired: 4 in, 1 out]
            n146 = property on="Property Node" class="Mod Admin"(reference=w327) -> ("Accessors:Module ID"=w326:i32)  [unwired: 1 in, 2 out]
            n147 = control-ref of="This VI"() -> (w328:refnum<vi>)
            n148 = call-dynamic "Delacor_lib_QMH_Release Message Queue.vi"("error in"=w341, "Message Queue"=w336) -> ("error out"=w340:errorcluster)  [unwired: 9 in]
            n149 = call "Handle Exit.vi"("Stop Argument"=w329, "Module Admin in"=w327, "VI reference"=w328) -> ("error out"=w339:errorcluster, "Wait for Stop?"=w330:bool)  [unwired: 7 in]
            n150 = Merge Errors(w340, w339) -> (w337:errorcluster)
            n151 = call "Error Reported.vi"("Error"=w337, "Module ID"=w326) -> ()  [unwired: 9 in, 1 out]
          }
          frame Default {
            # "'Default' case only runs if there is a message that isn't defined in any of the other cases.  Output a programming error."
            n152 = property on="Property Node" class="Mod Admin"(reference=w350) -> ("Accessors:Module ID"=w349:i32)  [unwired: 1 in, 2 out]
            n153 = call "Module Name--constant.vi"("Module ID"=w349) -> ("Module Name"=w343:string)  [unwired: 10 in]
            n154 = Format Into String(format string="The invalid message string \"%s\" was received in the Message Handling Loop for module \"%s\".", w344, w343) -> (resulting string=w346:string)  [unwired: 2 in, 1 out]
            n155 = call <vilib>:"Error Cluster From Error Code.vi"("show call chain? (False)"=TRUE, "error message (\"\")"=w346, "error code (0)"=1) -> ("error out"=w352:errorcluster)  [unwired: 6 in]
            n156 = Merge Errors(w353, w352) -> (w354:errorcluster)
          }
        }
        n157 = call-dynamic "Delacor_lib_QMH_Error Handler - Message Handling Loop.vi"("error in"=w216, "Message Queue in"=w207) -> ("dup error in"=w213:errorcluster)  [unwired: 8 in, 1 out]
      }
      n158 = while "DQMH_HELPER_LOOP" {
        shift-right: [w42] -> _
        shift-left: -1 -> [w41]
        shift-right: [w39] -> w22
        shift-left: w21 -> [w40]
        tunnel: w27 -> [w36]
        tunnel: w26 -> [w34]
        stop <- w38 stop-if-true
        w35 = "Helper Loop"  # DQMH_HELPER_LOOP_NAME
        # "Helper Loop"
        n159 = event "DQMH_HELPER_EVENT_STRUCTURE" shown="[2] <My Cloneable Module Request Events.Request a HL>: User Event" {
          selector: w40 -> [_ _ _]
          dyn-events: [_ _ _] -> w39
          timeout: w41 -> [_ _ _]
          tunnel: w41 -> [w43 w48 w53]
          tunnel: [w43 w48 w53] -> w42
          tunnel: [_ w45 _] -> w38
          tunnel: [_ errorcluster {"status"=FALSE, "code"=0, "source"=""} ("error constant") _] -> w37
          tunnel: w36 -> [_ _ _]
          tunnel: w34 -> [_ w46 w52]
          event Timeout {
            n160 = event-data() -> ()  [unwired: 1 in, 1 out]
          }
          event User Event {
            n161 = event-data() -> ("Module ID"=w44:i32)  [unwired: 1 in]
            n162 = call "Addressed to This Module.vi"("Module ID from Argument"=w44, "Module Admin"=w46) -> ("Addressed to this instance?"=w45:bool)  [unwired: 8 in, 1 out]
          }
          event User Event {
            # "Another Module called the \"Request a HL\" API Method."
            n163 = event-data() -> ("Module ID"=w51:i32, "String"=w49:string)  [unwired: 1 in]
            n164 = call "Addressed to This Module.vi"("Module ID from Argument"=w51, "Module Admin"=w52) -> ("Addressed to this instance?"=w50:bool)  [unwired: 8 in, 1 out]
            n165 = case shown="True" w50 {
              tunnel: w49 -> [_ _]
              frame False {
              }
              frame True {
              }
            }
          }
        }
        n166 = call-dynamic "Delacor_lib_QMH_Error Handler - Helper Loop.vi"("Error Debug"=w35, "error in"=w37, "Message Queue in"=w36) -> ()  [unwired: 7 in, 2 out]
      }
      n167 = Unregister For Events(event registration refnum=w22) -> ()  [unwired: 1 in, 1 out]
    }
    frame Error {
      n168 = call "Synchronize Caller Events.vi"("Module Admin"=w358) -> ("Module Admin out"=w357:refnum<class "Delacor_lib_QMH_Cloneable Module Admin.lvclass">)  [unwired: 9 in, 1 out]
      n169 = property on="Property Node" class="Mod Admin"(reference=w357) -> ("Accessors:Module ID"=w356:i32)  [unwired: 1 in, 2 out]
      n170 = call-dynamic "Delacor_lib_QMH_Release Message Queue.vi"("error in"=w364, "Message Queue"=w355) -> ("error out"=w363:errorcluster)  [unwired: 9 in]
      n171 = call "Module Name--constant.vi"("Module ID"=w356) -> ("Module Name"=w361:string)  [unwired: 10 in]
      n172 = Format Into String(format string="An error occurred during initialization. %s is no longer running.", w361) -> (resulting string=w359:string)  [unwired: 2 in, 1 out]
      n173 = call "Error Reported.vi"("Additional Information"=w359, "Error"=w363, "Module ID"=w356) -> ()  [unwired: 8 in, 1 out]
    }
  }
  n174 = Merge Errors(w18, w17) -> (w19:errorcluster)
  n175 = call "Close Module.vi"("error in"=w19, "Wait for stop?"=w4, "Module Admin in"=w6) -> ("error out"=w15:errorcluster, "External Launch"=w3:bool, "Module Admin out"=w5:refnum<class "Delacor_lib_QMH_Cloneable Module Admin.lvclass">)  [unwired: 6 in]
  n176 = Unregister For Events(event registration refnum=w10, error in=w15) -> (error out=w14:errorcluster)
  "error out" <- w14
  n177 = case "External Launch?" shown="True" w3 {
    tunnel: w14 -> [_ w365]
    frame False {
    }
    frame True {
      n178 = case shown="No Error" w365 {
        frame No Error {
          n179 = invoke class="VI" method="FP.Close"() -> ()  [unwired: 3 in, 3 out]
        }
        frame Error {
          n180 = disable-structure shown="Default" {
            frame condition #0 (active) {
              n181 = invoke class="VI" method="FP.Open"("Activate"=TRUE ("Activate?")) -> ()  [unwired: 4 in, 5 out]
            }
            frame condition #1 {
              # "Don't show panel on error if running inside a built EXE."
            }
          }
        }
      }
    }
  }
  n182 = local write "Module Admin"(w5) -> ()
